vi "Assert Equal Value and Type_Variant.vi"(4 "Execution time (s)":dbl=-1.0, 5 "Assert Only? (F)":bool, 6 "error code (1)":i32=1, 7 "Label":string, 8 "error in (no error)":errorcluster, 9 "Register with caller test (F)":bool, 10 "Actual":variant, 11 "Expected":variant) -> (0 "error out":errorcluster, 2 "Properties.Assert":refnum<class "Properties.Assert.lvclass">)   [LabVIEW 2013, in "Caraya.lvlib" / "Assert.lvclass"]
doc: "Generates an error if the input condition is not met.\n\nThis method compares the inputs after being cast to a Variant.\nAsserts TRUE if both type and value are equal.\nAsserts FALSE otherwise.\n\nex: Two integer inputs of equal value but of different type representation (U8 and I32) will assert FALSE."
uses:
  Assert.lvclass
  Properties.Assert/Properties.Assert.lvclass
  Properties/Properties.lvclass
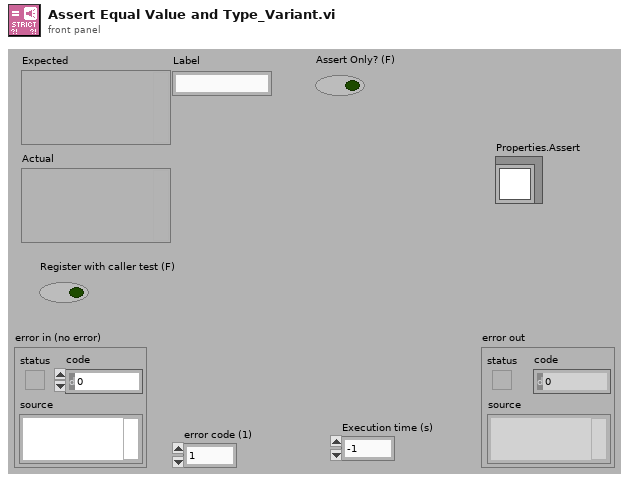
[diagram p1: front panel]
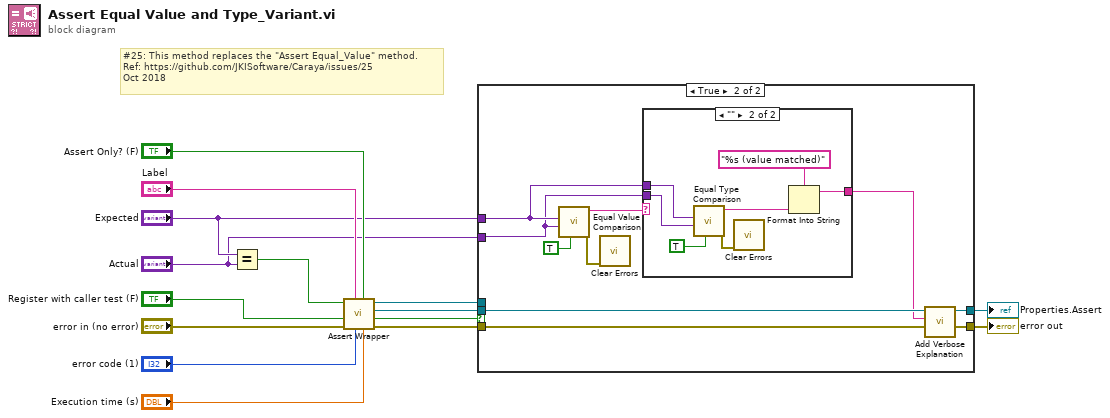
[diagram p0: block diagram]
diagram:
  # "#25: This method replaces the \"Assert Equal_Value\" method.\nRef: https://github.com/JKISoftware/Caraya/issues/25\nOct 2018"
  n1 = Equal?(x="Expected", y="Actual") -> (x = y?=w13:bool)
  n2 = call "Assert Wrapper.vi"("Execution time (s)"="Execution time (s)", "Assert Only? (F)"="Assert Only? (F)", "error code (1)"="error code (1)", "Label"="Label", "error in (no error)"="error in (no error)", "Register with caller test (F)"="Register with caller test (F)", "Assert?"=w13) -> ("error out"=w10:errorcluster, "Verbose"=w5:bool, "Properties.Assert"=w2:refnum<class "Properties.Assert.lvclass">, "Assert out"=w3:refnum<class "Assert.lvclass">)  [unwired: 1 in]
  n3 = case shown="True" w5 {
    tunnel: [w17 w20] -> w6
    tunnel: w3 -> [_ _]
    tunnel: w10 -> [w17 w21]
    tunnel: "Expected" -> [_ w27]
    tunnel: "Actual" -> [_ w26]
    tunnel: w2 -> [w16 w22]
    tunnel: [w16 w18] -> w1
    frame False {
    }
    frame True {
      n4 = call "Equal Value Comparison.vi"("verbose? (F)"=TRUE, "Actual"=w26, "Expected"=w27) -> ("error out"=w24:errorcluster, "Verbose output"=w23:string)  [unwired: 6 in, 1 out]
      n5 = call <vilib>:"Clear Errors.vi"("error in (no error)"=w24) -> ()  [unwired: 6 in, 1 out]
      n6 = case shown="\"\"" w23 {
        selector: w23 -> [w28 _]
        tunnel: [w28 w30] -> w19
        tunnel: w27 -> [_ w33]
        tunnel: w26 -> [_ w32]
        frame Default {
        }
        frame "" {
          n7 = call "Equal Type Comparison.vi"("verbose? (F)"=TRUE, "Actual"=w32, "Expected"=w33) -> ("error out"=w35:errorcluster, "Verbose output"=w31:string)  [unwired: 6 in, 1 out]
          n8 = call <vilib>:"Clear Errors.vi"("error in (no error)"=w35) -> ()  [unwired: 6 in, 1 out]
          n9 = Format Into String(format string="%s (value matched)", w31) -> (resulting string=w30:string)  [unwired: 2 in, 1 out]
        }
      }
      n10 = call "Add Verbose Explanation.vi"("error in (no error)"=w21, "Verbose Explanation"=w19, "Properties"=w22) -> ("error out"=w20:errorcluster, "Properties"=w18:refnum<class "Properties.Assert.lvclass">)  [unwired: 7 in]
    }
  }
  "error out" <- w6
  "Properties.Assert" <- w1
